vi "close.vi"(8 "error in":errorcluster, 11 "Modbus Slave runtime in":refnum<class "Modbus Module runtime.lvclass">) -> (0 "error out":errorcluster)   [LabVIEW 2015, in "Modbus Module runtime.lvclass"]
doc: "Provides an interface for terminating a module instance. While this interface performs no operations, a child should close and deallocate any open references or memory.Platypus Framework 1.0.1.65\nNI Systems Engineering - National Instruments"
uses:
  Modbus Module runtime.lvclass
  Modbus Module runtime.lvclass/Modbus Module runtime.ctl
  message to background process.ctl
  command enum.ctl
  <vilib>/NI/Tag Bus/table/data table.ctl
  modbus asynch.vi
  <vilib>/NI/Modbus Library/API/Modbus API.lvclass
  <vilib>/NI/Tag Bus/table/data table.lvlib
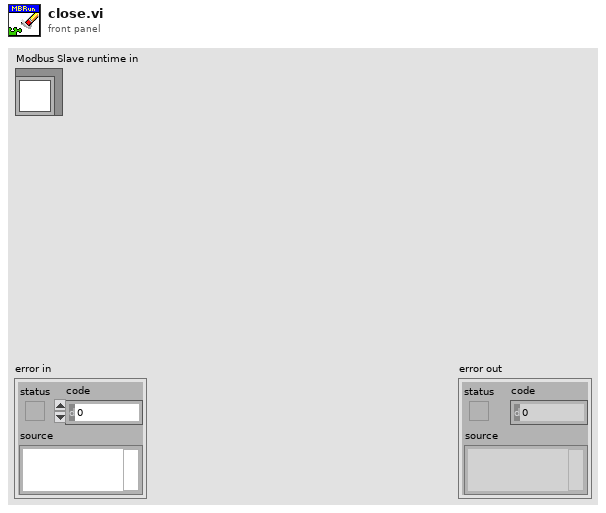
[diagram p1: front panel]
types:
  T1 = typedef "Modbus Module runtime.lvclass/asynch process references.ctl" = cluster{"commands":refnum<k33>, "input buffer":refnum<k33>, "output buffer":refnum<k33>, "asynch VI ref":variant, "original DVRs":refnum<data-value>[]}
  T2 = typedef "Modbus Module runtime.lvclass/message to background process.ctl" = cluster{"command enum":T3, "datapack":refnum<data-value>}
  T3 = typedef "Modbus Module runtime.lvclass/command enum.ctl" = enum16{"stop", "input", "output"}
  T4 = typedef "Modbus Module runtime.lvclass/response from background process.ctl" = cluster{"response enum":T5, "datapack":refnum<data-value>, "error code":i32}
  T5 = typedef "Modbus Module runtime.lvclass/response enum.ctl" = enum16{"exit", "return buffer", "error"}
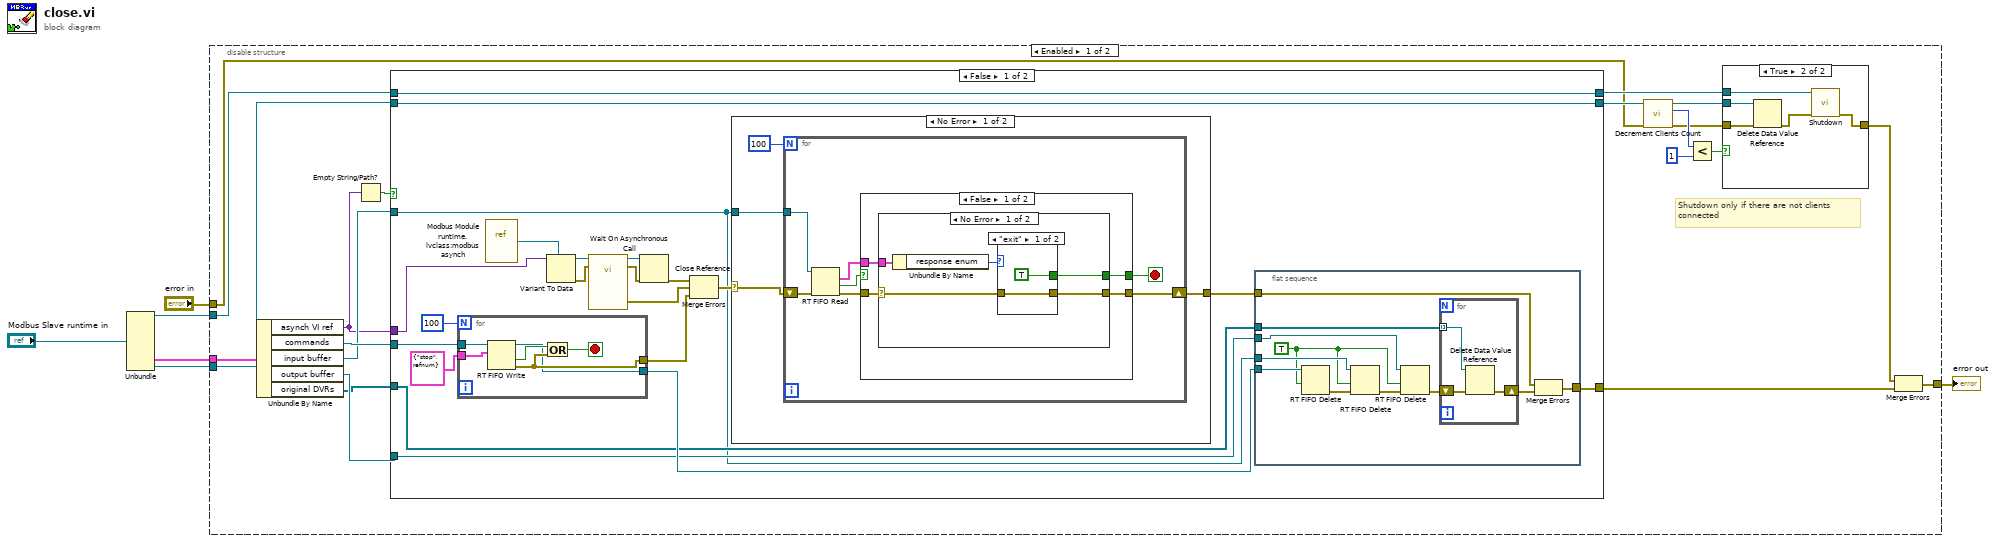
[diagram p0: block diagram]
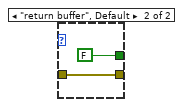
[diagram p3: hidden frame]
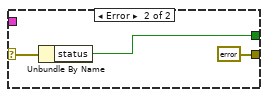
[diagram p4: hidden frame]
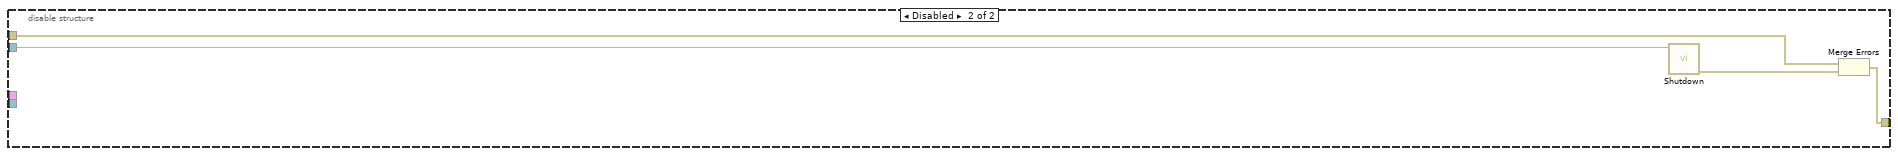
[diagram p8: hidden frame]
diagram:
  n1 = Unbundle("Modbus Slave runtime in") -> (w5:refnum<class "Modbus API.lvclass">, w4:T1, w1:refnum<data-value>)  [unwired: 5 out]
  n2 = disable-structure shown="Enabled" {
    disable-tunnel: w5 -> [w18 w107]
    disable-tunnel: w4 -> [w26 _]
    disable-tunnel: [w16 w109] -> w3
    disable-tunnel: "error in" -> [w13 w108]
    disable-tunnel: w1 -> [w15 _]
    frame Enabled {
      # "Shutdown only if there are not clients\nconnected"
      n3 = Unbundle By Name(w26) -> ("asynch VI ref"=w20:variant, "commands"=w25:refnum<k33>, "input buffer"=w22:refnum<k33>, "output buffer"=w24:refnum<k33>, "original DVRs"=w23:refnum<data-value>[])
      n4 = Empty String/Path?(string/path=w20) -> (empty?=w19:bool)
      n5 = case shown="False" w19 {
        tunnel: w25 -> [w53 _]
        tunnel: w24 -> [w41 _]
        tunnel: w23 -> [w40 _]
        tunnel: w22 -> [w37 _]
        tunnel: [w36 _] -> w21
        tunnel: w20 -> [w35 _]
        tunnel: w18 -> [w34 w105]
        tunnel: [w34 w105] -> w17
        tunnel: w15 -> [w33 w104]
        tunnel: [w33 w104] -> w14
        frame False {
          n6 = for {
            N: 100 -> [_]
            tunnel: w53 -> [w103]
            tunnel: T2 {"command enum"=enum."stop", "datapack"=refnum} ("element") -> [w102]
            tunnel: [w99] -> w43
            tunnel: [w98] -> w42
            stop <- w100 stop-if-true
            n7 = RT FIFO Write(0:w103, 1:w102) -> (8:w98:refnum<k33>, 10:w101:bool, 11:w99:errorcluster)  [unwired: 3 in, 1 out]
            n8 = Or(x=w101, y=w99) -> (x .or. y?=w100:bool)
          }
          n9 = vi-ref "Modbus Module runtime.lvclass:modbus asynch.vi"() -> (w50:refnum<vi>)
          n10 = Variant To Data(type=w50, Variant=w35) -> (data=w49:refnum<vi>, error out=w48:errorcluster)  [unwired: 1 in]
          n11 = call-by-ref "Wait On Asynchronous Call"(reference=w49, error in=w48) -> (reference out=w46:refnum<vi>, error out=w47:errorcluster, 0:"error out"=w44:errorcluster)  [unwired: 11 in]
          n12 = Close Reference(reference=w46, error in (no error)=w47) -> (error out=w45:errorcluster)
          n13 = Merge Errors(w45, w44, w43) -> (w39:errorcluster)
          n14 = case shown="No Error" w39 {
            selector: w39 -> [w70 w97]
            tunnel: [w68 w97] -> w38
            tunnel: w37 -> [w69 _]
            frame No Error {
              n15 = for {
                N: 100 -> [_]
                shift-right: [w72] -> w68
                shift-left: w70 -> [w78]
                tunnel: w69 -> [w77]
                stop <- w74 stop-if-true
                n16 = RT FIFO Read(0:w77, 3:w78) -> (9:w76:T4, 10:w75:bool, 11:w73:errorcluster)  [unwired: 2 in, 2 out]
                n17 = case shown="False" w75 {
                  selector: w75 -> [_ w96]
                  tunnel: w76 -> [w82 _]
                  tunnel: [w79 w96] -> w74
                  tunnel: w73 -> [w81 w95]
                  tunnel: [w80 w95] -> w72
                  frame False {
                    n18 = case shown="No Error" w81 {
                      selector: w81 -> [w85 w94]
                      tunnel: w82 -> [w87 _]
                      tunnel: [w84 errorcluster {"status"=FALSE, "code"=0, "source"=""} ("error IO")] -> w80
                      tunnel: [w83 w93] -> w79
                      frame No Error {
                        n19 = Unbundle By Name(w87) -> ("response enum"=w86:T5)
                        n20 = case shown="\"exit\"" w86 {
                          tunnel: w85 -> [w88 w91]
                          tunnel: [w88 w91] -> w84
                          tunnel: [TRUE FALSE] -> w83
                          frame "exit" {
                          }
                          frame "return buffer", Default {
                          }
                        }
                      }
                      frame Error {
                        n21 = Unbundle By Name(w94) -> ("status"=w93:bool)
                      }
                    }
                  }
                  frame True {
                  }
                }
              }
            }
            frame Error {
            }
          }
          n22 = flat-sequence {
            tunnel: w42 -> [w64]
            tunnel: w41 -> [w63]
            tunnel: w40 -> [w62]
            tunnel: w38 -> [w61]
            tunnel: w37 -> [w60]
            tunnel: [w59] -> w36
            frame #0 {
              w55 = TRUE ("force destroy? (F)")
              n23 = RT FIFO Delete(0:w64, 2:w55) -> (11:w58:errorcluster)  [unwired: 1 in]
              n24 = RT FIFO Delete(0:w60, 2:w55, 3:w58) -> (11:w57:errorcluster)
              n25 = RT FIFO Delete(0:w63, 2:w55, 3:w57) -> (11:w54:errorcluster)
              n26 = for {
                tunnel: w62 -> [w67] mode=indexing
                shift-right: [w66] -> w56
                shift-left: w54 -> [w65]
                n27 = Delete Data Value Reference(data value reference=w67, error in=w65) -> (error out=w66:errorcluster)  [unwired: 1 out]
              }
              n28 = Merge Errors(w61, w56) -> (w59:errorcluster)
            }
          }
        }
        frame True {
        }
      }
      n29 = call "Decrement Clients Count.vi"("error in (no error)"=w13, "Data Value Reference in"=w14) -> ("error out"=w8:errorcluster, "Clients count"=w12:i32, "Data Value Reference out"=w9:refnum<data-value>)  [unwired: 7 in]
      n30 = Less?(x=w12, y=1) -> (x < y?=w10:bool)
      n31 = case shown="True" w10 {
        tunnel: w17 -> [_ w32]
        tunnel: w9 -> [_ w31]
        tunnel: w8 -> [w27 w30]
        tunnel: [w27 w28] -> w7
        frame False {
        }
        frame True {
          n32 = Delete Data Value Reference(data value reference=w31, error in=w30) -> (error out=w29:errorcluster)  [unwired: 1 out]
          n33 = call-dynamic "Shutdown.vi"("error in"=w29, "Modbus instance in"=w32) -> ("error out"=w28:errorcluster)  [unwired: 9 in]
        }
      }
      n34 = Merge Errors(w7, w21) -> (w16:errorcluster)
    }
    frame Disabled {
      n35 = call-dynamic "Shutdown.vi"("Modbus instance in"=w107) -> ("error out"=w106:errorcluster)  [unwired: 10 in]
      n36 = Merge Errors(w108, w106) -> (w109:errorcluster)
    }
  }
  "error out" <- w3
